vi "query Start and Stop Frequency.vi"(8 "error in (no error)":errorcluster, 11 "Keysight 9020A in":refnum<class "Keysight 9020A.lvclass">) -> (0 "error out":errorcluster, 2 "Start/Stop Frequency(Hz)":T1 {"Stop" format="%#_6p"; "Start" format="%#_6p"}, 3 "Keysight 9020A out":refnum<class "Keysight 9020A.lvclass">)   [LabVIEW 2023, in "Spectrum Analyzer.lvlib" / "Keysight 9020A.lvclass"]
uses:
  Keysight 9020A.lvclass
  TYPE DEFINITION/TYPE Start and Stop Frequency.ctl
  Keysight 9020A.lvclass/Keysight 9020A.ctl
  Spectrum Analyzer.lvlib
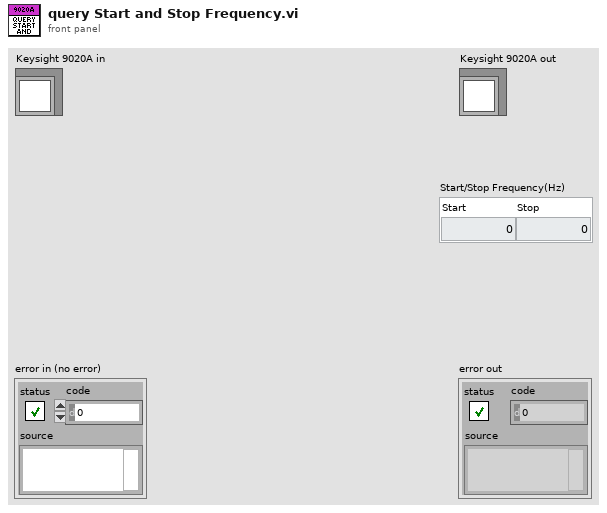
[diagram p1: front panel]
types:
  T1 = typedef "Spectrum Analyzer.lvlib/TYPE Start and Stop Frequency.ctl" = cluster{"Start":dbl, "Stop":dbl}
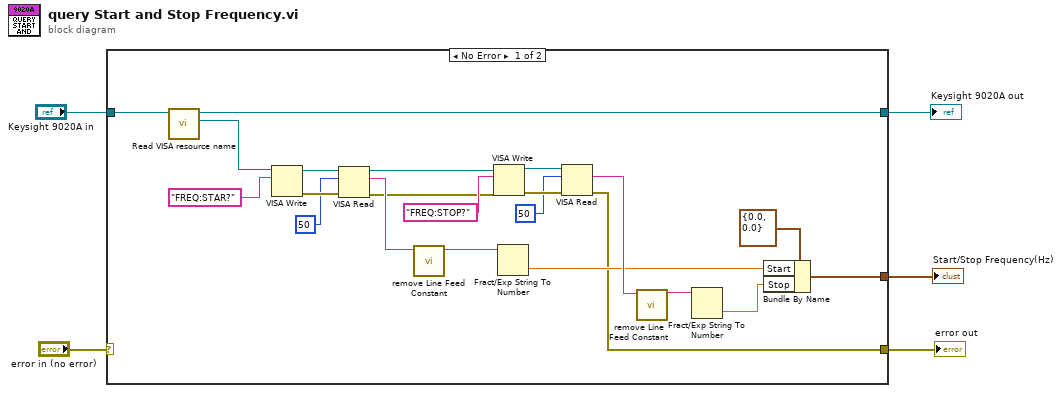
[diagram p0: block diagram]
diagram:
  n1 = case shown="No Error" "error in (no error)" {
    selector: "error in (no error)" -> [_ w28]
    tunnel: "Keysight 9020A in" -> [w27 w29]
    tunnel: [w26 w29] -> w4
    tunnel: [w7 w28] -> w2
    tunnel: [w6 _] -> w1
    frame No Error {
      n2 = call "Read VISA resource name.vi"("Keysight 9020A in"=w27) -> ("VISA resource name"=w8:refnum<visa-resource-name>, "Keysight 9020A out"=w26:refnum<class "Keysight 9020A.lvclass">)  [unwired: 8 in, 1 out]
      n3 = VISA Write(VISA resource name=w8, write buffer="FREQ:STAR?") -> (VISA resource name out=w23:refnum<visa-resource-name>, error out=w22:errorcluster)  [unwired: 1 in, 1 out]
      n4 = VISA Read(VISA resource name=w23, byte count=u32 50, error in (no error)=w22) -> (VISA resource name out=w19:refnum<visa-resource-name>, read buffer=w20:string, error out=w18:errorcluster)  [unwired: 1 out]
      n5 = call "remove Line Feed Constant.vi"("Input String"=w20) -> ("Line Feed Removed String"=w13:string)  [unwired: 10 in]
      n6 = VISA Write(VISA resource name=w19, write buffer="FREQ:STOP?", error in (no error)=w18) -> (VISA resource name out=w17:refnum<visa-resource-name>, error out=w16:errorcluster)  [unwired: 1 out]
      n7 = Fract/Exp String To Number(string=w13) -> (number=w11:dbl)  [unwired: 3 in, 1 out]
      n8 = VISA Read(VISA resource name=w17, byte count=u32 50, error in (no error)=w16) -> (read buffer=w14:string, error out=w7:errorcluster)  [unwired: 2 out]
      n9 = call "remove Line Feed Constant.vi"("Input String"=w14) -> ("Line Feed Removed String"=w10:string)  [unwired: 10 in]
      n10 = Fract/Exp String To Number(string=w10) -> (number=w9:dbl)  [unwired: 3 in, 1 out]
      n11 = Bundle By Name(cluster=T1 {"Start"=0.0, "Stop"=0.0} ("Start/Stop Frequency(Hz) 2"), "Start"=w11, "Stop"=w9) -> (w6:T1)
    }
    frame Error {
    }
  }
  "error out" <- w2
  "Keysight 9020A out" <- w4
  "Start/Stop Frequency(Hz)" <- w1
